vi "Merge Diff Images.vi"(7 "error in (no error)":errorcluster, 8 "ID":i32, 9 "Before = F | After = T?":bool, 10 "Diff PNG Files":path[](array[path])) -> (0 "error out":errorcluster)   [LabVIEW 2021, in "Graphical Diff.lvlib"]
uses:
  Graphical Diff.lvlib
  4bd7a358-025b-436a-b08a-e2c5914ece35.vi
  6fabf7ea-5db0-41f0-8f7d-caee261b24fd.vi
  <vilib>/numeric/Random Number (Range) I64.vi
  <vilib>/numeric/sub_Random U32.vi
  <vilib>/Comparison/Equal/Equal Functor/Equal Functor.lvclass
panel:
  out "colors":u32[](array[colorbox])
  out "merged picture":picture
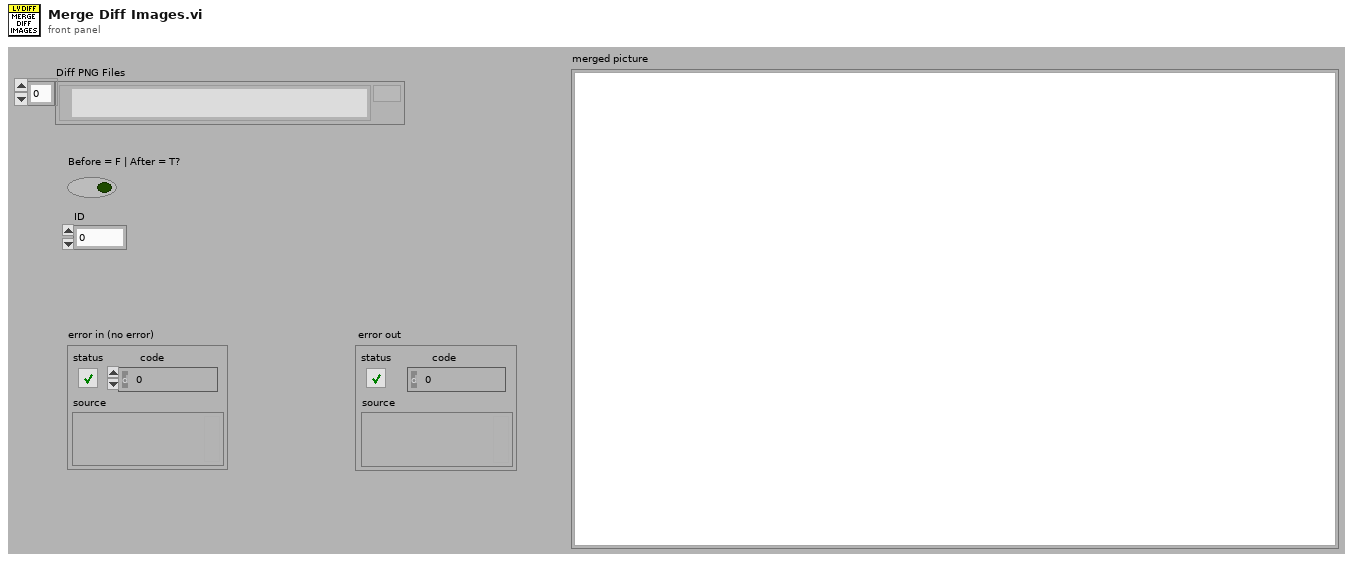
[diagram p1: front panel]
types:
  T1 = typedef "imagedata.ctl" = cluster{"image type":i32, "image depth":i32, "image":u8[], "mask":u8[], "colors":u32[], "Rectangle":cluster{"left":i16, "top":i16, "right":i16, "bottom":i16}}
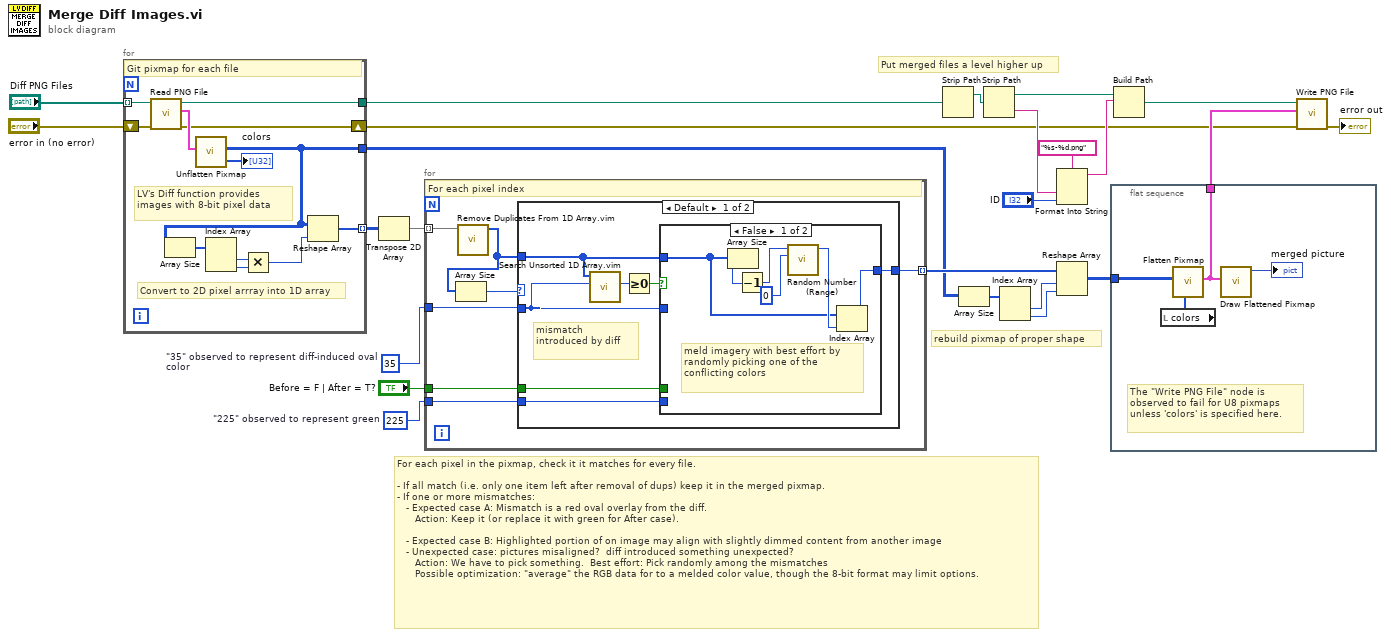
[diagram p0: block diagram]
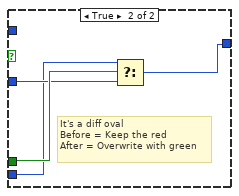
[diagram p2: hidden frame]
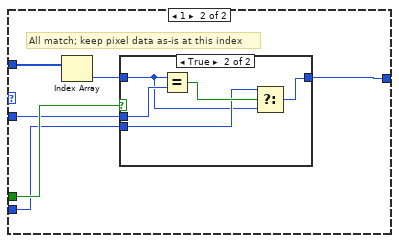
[diagram p3: hidden frame]
diagram:
  w10 = u8 225  # "225" observed to represent green
  w11 = u8 35  # "35" observed to represent diff-induced oval color
  # "Put merged files a level higher up"
  # "rebuild pixmap of proper shape"
  # "For each pixel in the pixmap, check it it matches for every file.\n\n- If all match (i.e. only one item left after removal of dups) keep it in the merged pixmap.\n- If one or more mismatches:\n   - Expected case A: Mismatch is a red oval overlay from the diff.\n      Action: Keep it (or replace it with green for After case).\n\n   - Expected case B: Highlighted portion of on image may align with slightly dimmed content from another image\n   - Unexpected case: pictures misaligned?  diff introduced something unexpected?\n      Action: We have to pick something.  Best effort: Pick randomly among the mismatches\n      Possible optimization: \"average\" the RGB data for to a melded color value, though the 8-bit format may limit options."
  n1 = for {
    tunnel: [w28] -> w18
    tunnel: [w35] -> w24
    tunnel: "Diff PNG Files" -> [w34] mode=indexing
    tunnel: [w33] -> w22 mode=indexing
    shift-right: [w25] -> w2
    shift-left: "error in (no error)" -> [w26]
    # "LV's Diff function provides images with 8-bit pixel data"
    # "Convert to 2D pixel arrray into 1D array"
    # "Git pixmap for each file"
    n2 = call <vilib>:"Read PNG File.vi"("error in (no error)"=w26, "path to PNG file"=w34) -> ("error out"=w25:errorcluster, "image data"=w36:T1, "path"=w35:path)  [unwired: 7 in]
    n3 = call <vilib>:"Unflatten Pixmap.vi"("image data"=w36) -> ("8-bit pixmap"=w28:u8[][], "colors"=→"colors":u32[])  [unwired: 4 in, 5 out]
    n4 = Array Size(array=w28) -> (size(s)=w32:i32[])
    n5 = Index Array(array=w32) -> (element #1=w30:i32, element #2=w31:i32)  [unwired: 2 in]
    n6 = Multiply(x=w30, y=w31) -> (x*y=w29:i32)
    n7 = Reshape Array(w28, w29) -> (w33:u8[])
  }
  n8 = Transpose 2D Array(2D array=w22) -> (transposed array=w21:u8[][])
  n9 = for {
    tunnel: w21 -> [w43] mode=indexing
    tunnel: [w40] -> w20 mode=indexing
    tunnel: "Before = F | After = T?" -> [w39]
    tunnel: w11 -> [w38]
    tunnel: w10 -> [w37]
    # "For each pixel index"
    n10 = call "Remove Duplicates From 1D Array.vim"("array"=w43) -> ("array with duplicates removed"=w41:u8[])  [unwired: 10 in]
    n11 = Array Size(array=w41) -> (size(s)=w42:i32)
    n12 = case shown="Default" w42 {
      tunnel: w41 -> [w49 w66]
      tunnel: [w50 w64] -> w40
      tunnel: w39 -> [w46 w65]
      tunnel: w38 -> [w45 w62]
      tunnel: w37 -> [w44 w61]
      frame Default {
        # "mismatch introduced by diff"
        n13 = call "Search Unsorted 1D Array.vim"("element"=w45, "unsorted 1D array"=w49) -> ("index of element"=w48:i32)  [unwired: 9 in]
        n14 = Greater Or Equal To 0?(x=w48) -> (x >= 0?=w47:bool)
        n15 = case shown="False" w47 {
          tunnel: [w54 w58] -> w50
          tunnel: w49 -> [w51 _]
          tunnel: w45 -> [_ w59]
          tunnel: w46 -> [_ w60]
          tunnel: w44 -> [_ w57]
          frame False {
            # "meld imagery with best effort by randomly picking one of the conflicting colors"
            n16 = Array Size(array=w51) -> (size(s)=w56:i32)
            n17 = Decrement(x=w56) -> (x-1=w53:i32)
            n18 = call-poly <vilib>:"Random Number (Range).vi"("lower bound (-100)"=i64 0, "upper bound (100)"=w53) -> ("number"=w55:i64)  [unwired: 9 in]
            n19 = Index Array(array=w51, index=w55) -> (element=w54:u8)
          }
          frame True {
            # "It's a diff oval\nBefore = Keep the red\nAfter = Overwrite with green"
            n20 = Select(t=w57, s=w60, f=w59) -> (s? t:f=w58:u8)
          }
        }
      }
      frame 1 {
        # "All match; keep pixel data as-is at this index"
        n21 = Index Array(array=w66) -> (element=w63:u8)  [unwired: 1 in]
        n22 = case shown="True" w65 {
          tunnel: [w67 w68] -> w64
          tunnel: w63 -> [w67 w69]
          tunnel: w62 -> [_ w72]
          tunnel: w61 -> [_ w70]
          frame False {
          }
          frame True {
            n23 = Equal?(x=w69, y=w72) -> (x = y?=w71:bool)
            n24 = Select(t=w70, s=w71, f=w69) -> (s? t:f=w68:u8)
          }
        }
      }
    }
  }
  n25 = Strip Path(path=w24) -> (stripped path=w13:path)  [unwired: 1 out]
  n26 = Array Size(array=w18) -> (size(s)=w19:i32[])
  n27 = Strip Path(path=w13) -> (stripped path=w12:path, name=w8:string)
  n28 = Index Array(array=w19) -> (element #1=w17:i32, element #2=w16:i32)  [unwired: 2 in]
  n29 = Format Into String(format string="%s-%d.png", w8, "ID") -> (resulting string=w6:string)  [unwired: 2 in, 1 out]
  n30 = Reshape Array(w20, w17, w16) -> (w15:u8[][])
  n31 = flat-sequence {
    tunnel: w15 -> [w75]
    tunnel: [w73] -> w4
    frame #0 {
      # "The \"Write PNG File\" node is observed to fail for U8 pixmaps unless 'colors' is specified here."
      n32 = local read "colors"() -> (w74:u32[])
      n33 = call <vilib>:"Flatten Pixmap.vi"("colors"=w74, "8-bit pixmap"=w75) -> ("image data"=w73:T1)  [unwired: 9 in]
      n34 = call <vilib>:"Draw Flattened Pixmap.vi"("image data"=w73) -> ("new picture"=→"merged picture":picture)  [unwired: 8 in]
    }
  }
  n35 = Build Path(base path=w12, name or relative path=w6) -> (appended path=w3:path)
  n36 = call <vilib>:"Write PNG File.vi"("error in (no error)"=w2, "image data"=w4, "path to PNG file"=w3) -> ("error out"=→"error out":errorcluster)  [unwired: 7 in, 1 out]
